vi "FuncVI_Sub - xxGraph - Launcher.vi"(7 "Master VI Refnum":refnum<vi>, 8 "error in":errorcluster, 9 "left-top corner":cluster{"x":i16, "y":i16}={"x"=-1, "y"=-1}, 10 "win name":string, 11 "data":string) -> (0 "error out":errorcluster)   [LabVIEW 2021]
doc: "::: CalcExpress Toolkit :::\nCopyright (c) 2000-2026 Konstantin Shifershteyn. All rights reserved."
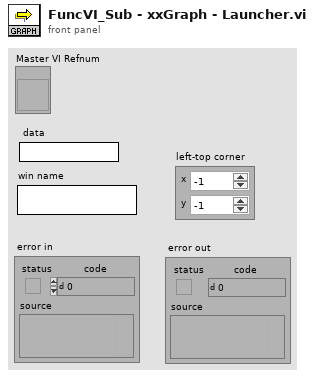
[diagram p1: front panel]
types:
  T1 = enum32{"Invalid", "Standard", "Closed", "Hidden", "Minimized", "Maximized"}
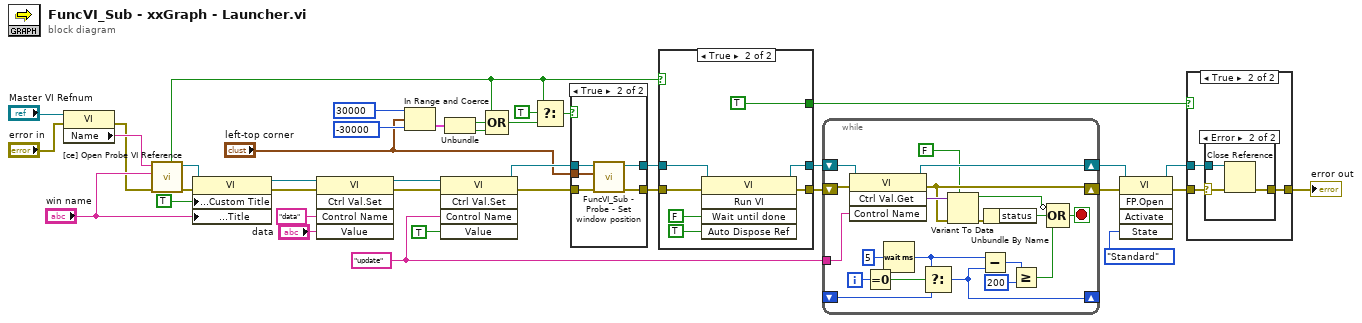
[diagram p0: block diagram]
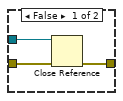
[diagram p2: hidden frame]
diagram:
  w21 = "update" ("Control Name")
  n1 = property class="VI"(reference="Master VI Refnum", error in="error in") -> (error out=w14:errorcluster, "Name"=w15:string)  [unwired: 1 out]
  n2 = call "[ce] Open Probe VI Reference.vi"("error in"=w14, "VI instance name"="win name", "master VI name"=w15) -> ("error out"=w31:errorcluster, "vi refnum"=w30:refnum<vi>, "new window?"=w3:bool)  [unwired: 6 in]
  n3 = property class="VI"(reference=w30, error in=w31, "Front Panel Window:Custom Title"=TRUE ("Front Panel.CustomTitle"), "Front Panel Window:Title"="win name") -> (reference out=w33:refnum<vi>, error out=w32:errorcluster)
  n4 = invoke class="VI" method="Ctrl Val.Set"(reference=w33, error in=w32, "Control Name"="data", "Value"="data") -> (reference out=w36:refnum<vi>, error out=w35:errorcluster)  [unwired: 1 in, 3 out]
  n5 = In Range and Coerce(upper limit=i16 30000 ("x"), x="left-top corner", lower limit=i16 -30000 ("x")) -> (In Range?=w8:cluster{"x":bool, "y":bool})  [unwired: 1 out]
  n6 = invoke class="VI" method="Ctrl Val.Set"(reference=w36, error in=w35, "Control Name"=w21, "Value"=TRUE) -> (reference out=w27:refnum<vi>, error out=w28:errorcluster)  [unwired: 1 in, 3 out]
  n7 = Unbundle(w8) -> ("x"=w6:bool, "y"=w5:bool)
  n8 = Compound Arithmetic op=OR(w3, w6, w5) -> (w4:bool)
  n9 = Select(t=w3, s=TRUE, f=w4) -> (s? t:f=w2:bool)
  n10 = case shown="True" w2 {
    tunnel: w28 -> [w41 w46]
    tunnel: w27 -> [w40 w45]
    tunnel: [w41 w44] -> w26
    tunnel: [w40 w43] -> w25
    tunnel: "left-top corner" -> [_ w42]
    frame False {
    }
    frame True {
      n11 = call "FuncVI_Sub - Probe - Set window position.vi"("error in"=w46, "left-top corner"=w42, "VI RefNum"=w45) -> ("error out"=w44:errorcluster, "dup VI Refnum"=w43:refnum<vi>)  [unwired: 7 in]
    }
  }
  n12 = case shown="True" w3 {
    tunnel: [w48 w53] -> w24
    tunnel: [w47 w54] -> w20
    tunnel: w25 -> [w48 w51]
    tunnel: w26 -> [w47 w52]
    tunnel: [_ TRUE] -> w11
    frame False {
    }
    frame True {
      n13 = invoke class="VI" method="Run VI"(reference=w51, error in=w52, "Wait until done"=FALSE, "Auto Dispose Ref"=TRUE ("Auto Dispose Reference")) -> (reference out=w53:refnum<vi>, error out=w54:errorcluster)  [unwired: 1 in, 3 out]
    }
  }
  n14 = while {
    shift-right: [w73] -> w22
    shift-left: w24 -> [w75]
    shift-right: [w60] -> w23
    shift-left: w20 -> [w74]
    shift-right: [w56] -> _
    shift-left: _ -> [w63]
    tunnel: w21 -> [w66]
    i -> [w65]
    stop <- w71 stop-if-true
    n15 = invoke class="VI" method="Ctrl Val.Get"(reference=w75, error in=w74, "Control Name"=w66) -> (reference out=w73:refnum<vi>, error out=w60:errorcluster, "Get Control Value Variant"=w61:variant)  [unwired: 1 in, 1 out]
    n16 = Equal To 0?(x=w65) -> (x = 0?=w62:bool)
    n17 = Wait (ms)(milliseconds to wait=u32 5) -> (millisecond timer value=w64:u32)
    n18 = Select(t=w64, s=w62, f=w63) -> (s? t:f=w56:u32)
    n19 = Variant To Data(error in=w60, type=FALSE, Variant=w61) -> (data=w57:bool, error out=w58:errorcluster)
    n20 = Subtract(x=w64, y=w56) -> (x-y=w69:u32)
    n21 = Unbundle By Name(w58) -> ("status"=w72:bool)
    n22 = Greater Or Equal?(x=w69, y=u32 200) -> (x >= y?=w67:bool)
    n23 = Compound Arithmetic op=OR(invert w57, w72, w67) -> (w71:bool)
  }
  n24 = invoke class="VI" method="FP.Open"(reference=w22, error in=w23, "State"=T1."Standard") -> (reference out=w39:refnum<vi>, error out=w12:errorcluster)  [unwired: 2 in, 3 out]
  n25 = case shown="True" w11 {
    tunnel: w39 -> [w78 w81]
    tunnel: [w76 w80] -> w37
    tunnel: w12 -> [w77 w79]
    frame False {
      n26 = Close Reference(reference=w78, error in (no error)=w77) -> (error out=w76:errorcluster)
    }
    frame True {
      n27 = case shown="Error" w79 {
        selector: w79 -> [w82 w83]
        tunnel: w81 -> [_ w85]
        tunnel: [w82 w84] -> w80
        frame No Error {
        }
        frame Error {
          n28 = Close Reference(reference=w85, error in (no error)=w83) -> (error out=w84:errorcluster)
        }
      }
    }
  }
  "error out" <- w37
